vi "VIH ProjFile - Path Array - Write.vi"(8 "error in":errorcluster, 9 "Paths":path[](array[path]), 10 "Property Name":string, 11 "XML Parent Item":refnum<k20>) -> (0 "error out":errorcluster, 3 "dup XML Parent Item":refnum<k20>)   [LabVIEW 2014]
doc: "::: VI Helpeks :::\nCopyright (c) 2000-2026 Konstantin Shifershteyn. All rights reserved."
uses:
  <vilib>/xml/Close Reference(Node).vi
  <resource>/objmgr/DOMUserDefRef.rc
  <vilib>/xml/NI_XML.lvlib
panel:
  # "VI Helpeks\nCopyright (c) 2012-2026 Konstantin Shifershteyn"
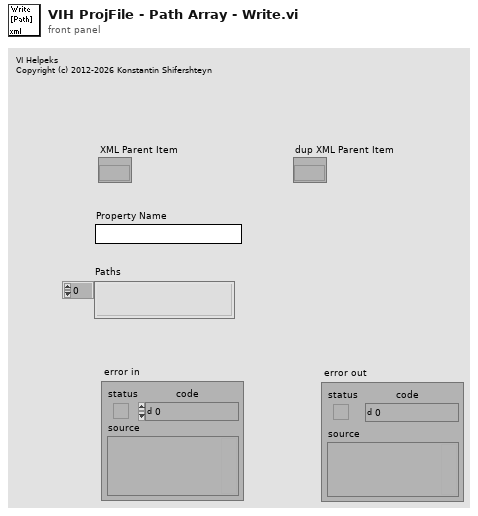
[diagram p1: front panel]
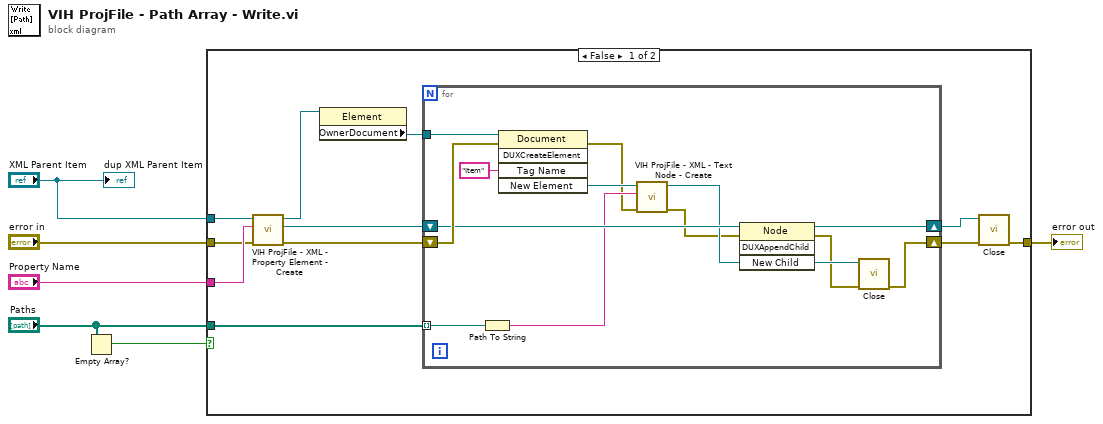
[diagram p0: block diagram]
diagram:
  n1 = Empty Array?(array="Paths") -> (empty?=w1:bool)
  n2 = case shown="False" w1 {
    tunnel: [w7 w31] -> w6
    tunnel: "XML Parent Item" -> [w10 _]
    tunnel: "Property Name" -> [w15 _]
    tunnel: "Paths" -> [w16 _]
    tunnel: "error in" -> [w9 w31]
    frame False {
      n3 = call "VIH ProjFile - XML - Property Element - Create.vi"("error in"=w9, "Property Name"=w15, "XML Parent Item"=w10) -> ("error out"=w13:errorcluster, "New Child"=w14:refnum<k20>, "dup XML Parent Item"=w11:refnum<k20>)  [unwired: 6 in]
      n4 = property class="Element"(reference=w11) -> ("OwnerDocument"=w12:refnum<k20>)  [unwired: 1 in, 2 out]
      n5 = for {
        shift-right: [w25] -> w8
        shift-left: w13 -> [w28]
        tunnel: w12 -> [w29]
        shift-right: [w26] -> w17
        shift-left: w14 -> [w27]
        tunnel: w16 -> [w24] mode=indexing
        n6 = Path To String(path=w24) -> (string=w22:string)
        n7 = invoke class="Document" method="DUXCreateElement"(reference=w29, error in=w28, "Tag Name"="Item") -> (error out=w19:errorcluster, "New Element"=w23:refnum<k20>)  [unwired: 2 in, 3 out]
        n8 = call "VIH ProjFile - XML - Text Node - Create.vi"("error in"=w19, "Data"=w22, "XML Parent Item"=w23) -> ("error out"=w18:errorcluster, "dup XML Parent Item"=w21:refnum<k20>)  [unwired: 7 in]
        n9 = invoke class="Node" method="DUXAppendChild"(reference=w27, error in=w18, "New Child"=w21) -> (reference out=w26:refnum<k20>, error out=w20:errorcluster)  [unwired: 1 in, 2 out]
        n10 = call-poly <vilib>:"Close.vi"("error in (no error)"=w20, "node"=w21) -> ("error out"=w25:errorcluster)  [unwired: 7 in]
      }
      n11 = call-poly <vilib>:"Close.vi"("error in (no error)"=w8, "node"=w17) -> ("error out"=w7:errorcluster)  [unwired: 7 in]
    }
    frame True {
    }
  }
  "error out" <- w6
  "dup XML Parent Item" <- "XML Parent Item"
